vi "LinearSystemSim_setInput.vi"(9 "Battery_Volts":dbl=12.0, 10 "Input":T1, 11 "in LinearSystemSim":T2) -> (0 "Size Coerced":bool, 3 "out LinearSystemSim":T2)   [LabVIEW 2019, in "Trajectory_Library.lvlib"]
doc: "Sets the system inputs (usually voltages).\n \nInputs:\n - LinearSystemSim -- Data cluster\n - Input -- The system inputs (u).\n - BatteryVolts -- Current battery voltage (volts)\n\nOutputs:\n - OutLinearSystemSim -- Updated data cluster\n - SizeCoerced -- If TRUE, an error occured. Execution may continue."
uses:
  Trajectory_Library.lvlib
  TypeDef/LINEAR_SYSTEM_SIM.ctl
  TypeDef/LINEAR_SYSTEM.ctl
  <vilib>/Analysis/Matrix/Datatypes/RealMatrix.ctl
  MatBuilder_Create.vi
  <vilib>/Analysis/Matrix/NI_Matrix.lvlib
panel:
  # "<States, 1>"
  # "<Outputs, 1>"
  # "<Inputs, 1>"
  # "<Outputs, 1>"
  # "<States,States>"
  # "<States,Inputs>"
  # "<Outputs,States>"
  # "<Outputs,Inputs>"
  # "<States, 1>"
  # "<Outputs, 1>"
  # "<Inputs, 1>"
  # "<Outputs, 1>"
  # "<States,States>"
  # "<States,Inputs>"
  # "<Outputs,States>"
  # "<Outputs,Inputs>"
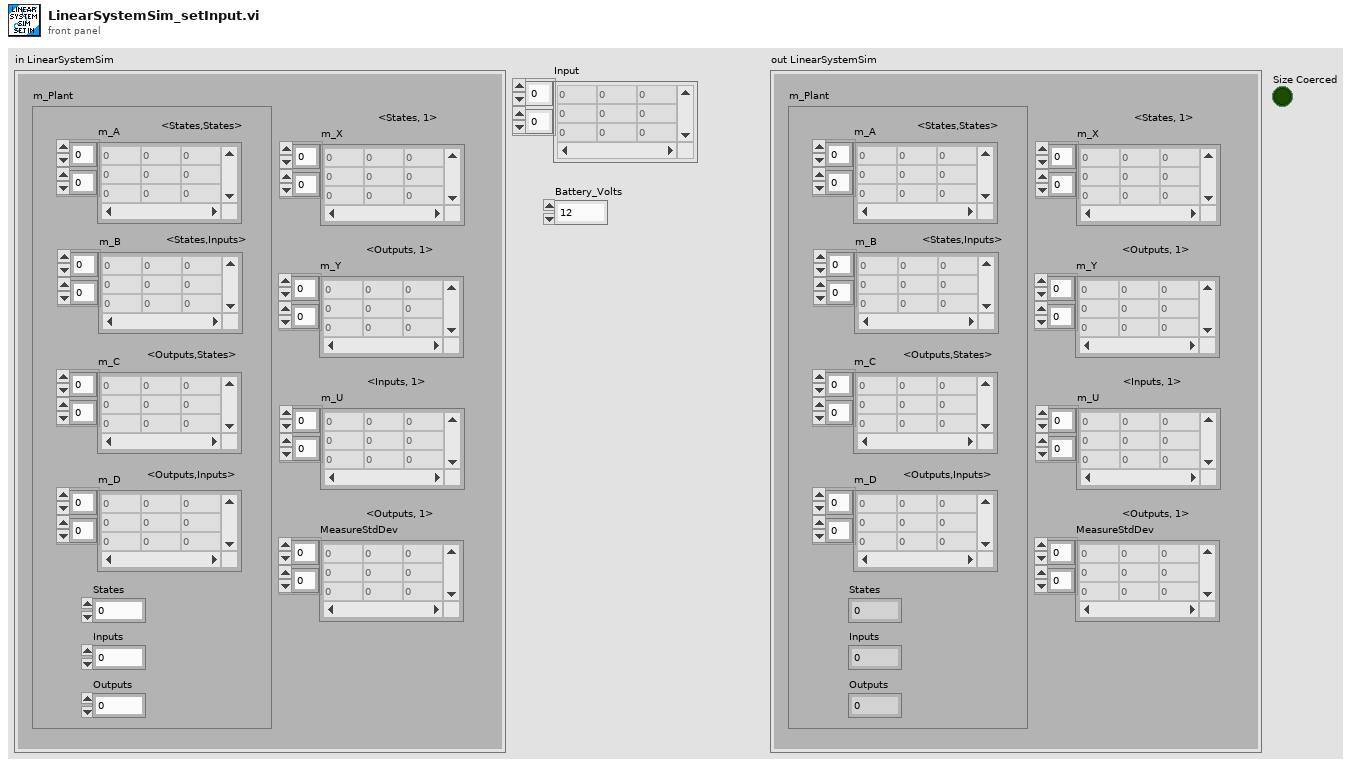
[diagram p1: front panel]
types:
  T1 = typedef "NI_Matrix.lvlib/RealMatrix.ctl" = dbl[][]
  T2 = typedef "Trajectory_Library.lvlib/LINEAR_SYSTEM_SIM.ctl" = cluster{"m_Plant":T3, "m_X":T1, "m_Y":T1, "m_U":T1, "MeasureStdDev":T1}
  T3 = typedef "Trajectory_Library.lvlib/LINEAR_SYSTEM.ctl" = cluster{"m_A":T1, "m_B":T1, "m_C":T1, "m_D":T1, "States":i32, "Inputs":i32, "Outputs":i32}
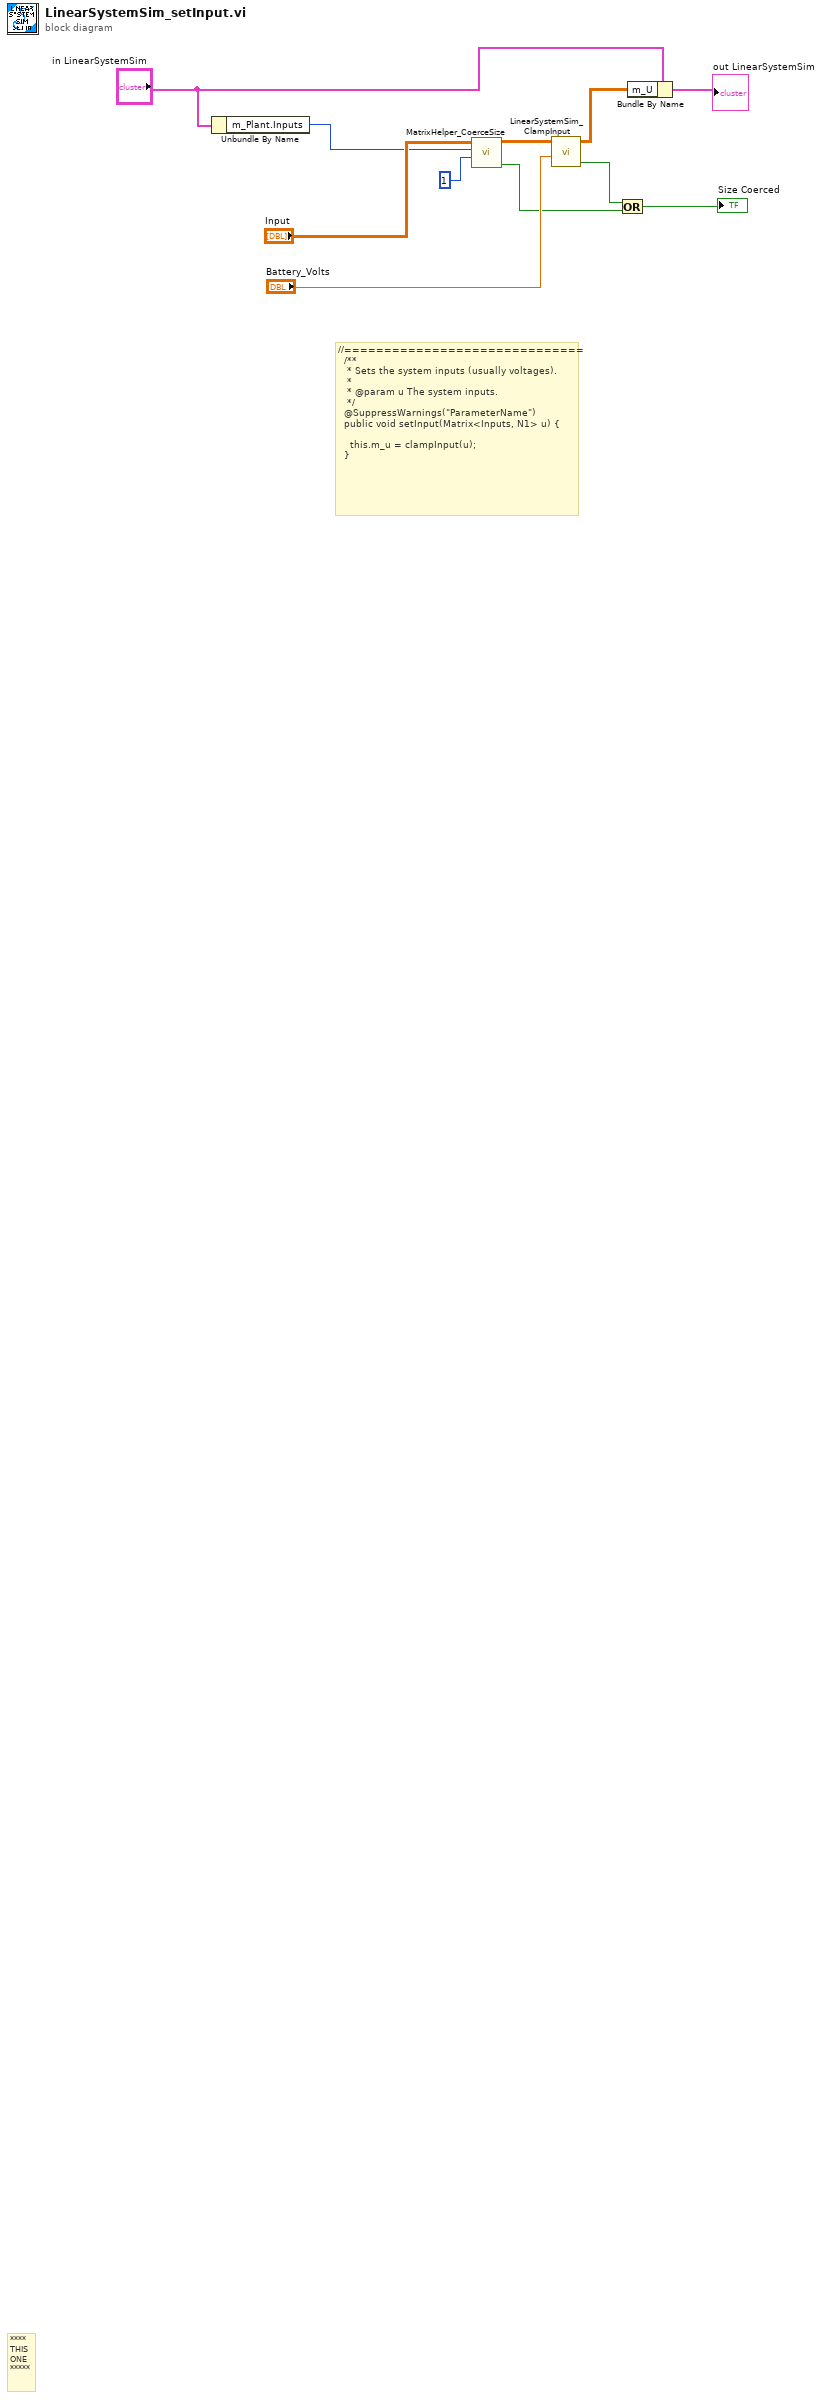
[diagram p0: block diagram]
diagram:
  # "//==============================\n  /**\n   * Sets the system inputs (usually voltages).\n   *\n   * @param u The system inputs.\n   */\n  @SuppressWarnings(\"ParameterName\")\n  public void setInput(Matrix<Inputs, N1> u) {\n\n    this.m_u = clampInput(u);\n  }"
  # "****\nTHIS\nONE\n*****"
  n1 = Unbundle By Name("in LinearSystemSim") -> ("m_Plant.Inputs"=w9:i32)
  n2 = call "MatrixHelper_CoerceSize.vi"("Columns"=1, "Rows"=w9, "input matrix"="Input") -> ("Coerced"=w1:bool, "output matrix"=w3:T1)  [unwired: 7 in]
  n3 = call "LinearSystemSim_ClampInput.vi"("Battery_Volts"="Battery_Volts", "Input"=w3) -> ("Size Coerced"=w2:bool, "ClampedInput"=w4:T1)  [unwired: 8 in]
  n4 = Or(x=w2, y=w1) -> (x .or. y?=→"Size Coerced":bool)
  n5 = Bundle By Name(cluster="in LinearSystemSim", "m_U"=w4) -> (→"out LinearSystemSim":T2)
